vi "Add content to Engine library.vi"(6 "Project Name":string, 8 "error in":errorcluster, 9 "Project Root":path, 10 "CD Wizard - Internal Data":T1, 11 "CD Template":refnum<class "NIVS_CD Template.lvclass">) -> (0 "error out":errorcluster)   [LabVIEW 2020, in "NIVS_CD Template.lvclass"]
doc: "Add all virtual folders and VIs to the Engine library."
uses:
  NIVS_CD Template.lvclass
  NIVS_Consolidated_CDW_MetaDataObj/Internal data.ctl
  NIVS_Consolidated_CDW_MetaDataObj/CD Engine lvlib.ctl
  NIVS_Consolidated_CDW_MetaDataObj/Add Item - Type.ctl
  NIVS_CD Template.lvclass/NIVS_CD Template.ctl
  NIVS_Consolidated_CDW_MetaDataObj/NIVS_Consolidated_CDW_MetaDataObj.lvclass
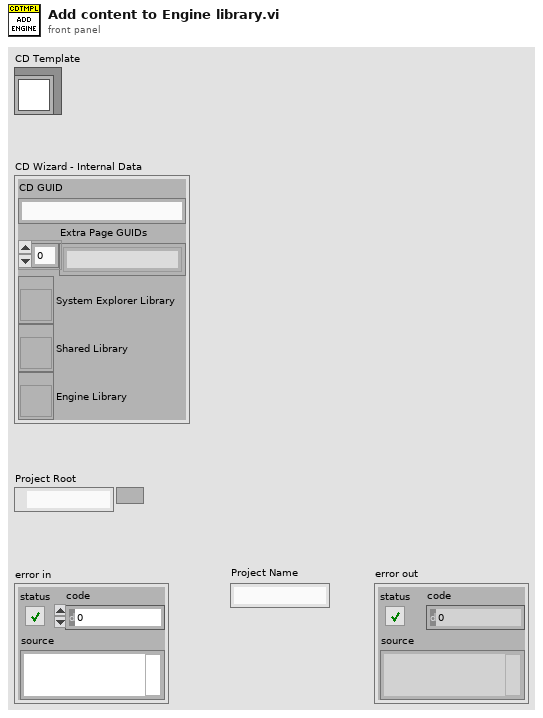
[diagram p1: front panel]
types:
  T1 = typedef "NIVS_Consolidated_CDW_MetaDataObj.lvclass/Internal data.ctl" = cluster{"CD GUID":string, "Extra Page GUIDs":string[], "System Explorer Library":refnum<vi>, "Shared Library":refnum<vi>, "Engine Library":refnum<vi>}
  T2 = typedef "NIVS_Consolidated_CDW_MetaDataObj.lvclass/CD Engine lvlib.ctl" = enum16{"LibraryFileName", "LibraryFolderName", "Engine.FolderName", "Engine.Init.FolderName", "Engine.Run.FolderName", "Engine.Shutdown.FolderName", "Types.FolderName", "Engine.RT Driver VI.TemplatePath", "Engine.RT Driver VI.FileName", "Engine.PPL.RT Driver VI_InlineAsync.FileName", "Engine.RTStateVariables.Name", "Engine.PPL.RTStateVariables.Name", "Engine.RTStateVariables.Name.NoExtension", "Engine.Async.NameExtension", "Engine.Async.TemplateName", "Engine.PPL.Async.TemplateName", "Engine.PPL.Async.InitVSGlobals.Name", "Engine.PPL.RT Driver VI_Inline.FileName", "Engine.LaunchCommandLoop.Name", "Engine.CommandLoop.Name"}
  T3 = typedef "NIVS_Consolidated_CDW_MetaDataObj.lvclass/Add Item - Type.ctl" = string
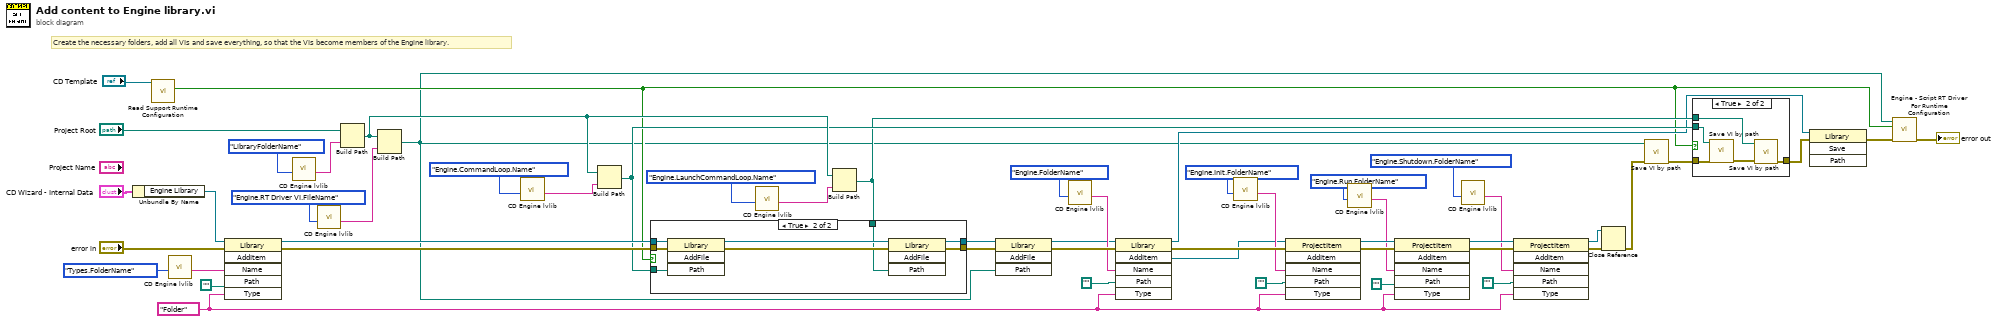
[diagram p0: block diagram]
diagram:
  w21 = T3 "Folder" ("Add Item - Type")
  # "Create the necessary folders, add all VIs and save everything, so that the VIs become members of the Engine library."
  n1 = Unbundle By Name("CD Wizard - Internal Data") -> ("Engine Library"=w33:refnum<vi>)
  n2 = call "Read Support Runtime Configuration.vi"("NIVS_CD Template in"="CD Template") -> ("Support Runtime Configuration"=w4:bool)  [unwired: 8 in, 2 out]
  n3 = call "CD Engine lvlib.vi"("Action"=CD_Engine_lvlib."Types.FolderName") -> ("Output"=w40:string)  [unwired: 10 in]
  n4 = invoke class="Library" method="AddItem"(reference=w33, error in="error in", "Name"=w40, "Path"=path "", "Type"=w21) -> (reference out=w36:refnum<vi>, error out=w51:errorcluster)  [unwired: 1 in, 4 out]
  n5 = call "CD Engine lvlib.vi"("Action"=CD_Engine_lvlib."LibraryFolderName") -> ("Output"=w34:string)  [unwired: 10 in]
  n6 = call "CD Engine lvlib.vi"("Action"=CD_Engine_lvlib."Engine.RT Driver VI.FileName") -> ("Output"=w35:string)  [unwired: 10 in]
  n7 = Build Path(base path="Project Root", name or relative path=w34) -> (appended path=w8:path)
  n8 = Build Path(base path=w8, name or relative path=w35) -> (appended path=w1:path)
  n9 = call "CD Engine lvlib.vi"("Action"=CD_Engine_lvlib."Engine.CommandLoop.Name") -> ("Output"=w11:string)  [unwired: 10 in]
  n10 = Build Path(base path=w8, name or relative path=w11) -> (appended path=w7:path)
  n11 = call "CD Engine lvlib.vi"("Action"=CD_Engine_lvlib."Engine.LaunchCommandLoop.Name") -> ("Output"=w10:string)  [unwired: 10 in]
  n12 = Build Path(base path=w8, name or relative path=w10) -> (appended path=w6:path)
  n13 = case shown="True" w4 {
    tunnel: w51 -> [w56 w64]
    tunnel: w7 -> [_ w61]
    tunnel: w6 -> [_ w59]
    tunnel: [w55 w58] -> w3
    tunnel: [w56 w62] -> w43
    tunnel: w36 -> [w55 w57]
    frame False {
    }
    frame True {
      n14 = invoke class="Library" method="AddFile"(reference=w57, error in=w64, "Path"=w61) -> (reference out=w60:refnum<vi>, error out=w63:errorcluster)  [unwired: 1 in, 2 out]
      n15 = invoke class="Library" method="AddFile"(reference=w60, error in=w63, "Path"=w59) -> (reference out=w58:refnum<vi>, error out=w62:errorcluster)  [unwired: 1 in, 2 out]
    }
  }
  n16 = invoke class="Library" method="AddFile"(reference=w3, error in=w43, "Path"=w1) -> (reference out=w2:refnum<vi>, error out=w42:errorcluster)  [unwired: 1 in, 2 out]
  n17 = call "CD Engine lvlib.vi"("Action"=CD_Engine_lvlib."Engine.FolderName") -> ("Output"=w31:string)  [unwired: 10 in]
  n18 = invoke class="Library" method="AddItem"(reference=w2, error in=w42, "Name"=w31, "Path"=path "", "Type"=w21) -> (reference out=w5:refnum<vi>, error out=w50:errorcluster, "AddItem"=w30:refnum<vi>)  [unwired: 1 in, 3 out]
  n19 = call "CD Engine lvlib.vi"("Action"=CD_Engine_lvlib."Engine.Init.FolderName") -> ("Output"=w37:string)  [unwired: 10 in]
  n20 = invoke class="ProjectItem" method="AddItem"(reference=w30, error in=w50, "Name"=w37, "Path"=path "", "Type"=w21) -> (reference out=w29:refnum<vi>, error out=w49:errorcluster)  [unwired: 1 in, 4 out]
  n21 = call "CD Engine lvlib.vi"("Action"=CD_Engine_lvlib."Engine.Run.FolderName") -> ("Output"=w28:string)  [unwired: 10 in]
  n22 = invoke class="ProjectItem" method="AddItem"(reference=w29, error in=w49, "Name"=w28, "Path"=path "", "Type"=w21) -> (reference out=w25:refnum<vi>, error out=w48:errorcluster)  [unwired: 1 in, 4 out]
  n23 = call "CD Engine lvlib.vi"("Action"=CD_Engine_lvlib."Engine.Shutdown.FolderName") -> ("Output"=w24:string)  [unwired: 10 in]
  n24 = invoke class="ProjectItem" method="AddItem"(reference=w25, error in=w48, "Name"=w24, "Path"=path "", "Type"=w21) -> (reference out=w23:refnum<vi>, error out=w53:errorcluster)  [unwired: 1 in, 4 out]
  n25 = Close Reference(reference=w23, error in (no error)=w53) -> (error out=w52:errorcluster)
  n26 = call "Save VI by path.vi"("error in (no error)"=w52, "VI path"=w1) -> ("error out"=w47:errorcluster)  [unwired: 9 in]
  n27 = case shown="True" w4 {
    tunnel: w47 -> [w65 w70]
    tunnel: [w65 w68] -> w46
    tunnel: w7 -> [_ w67]
    tunnel: w6 -> [_ w66]
    frame False {
    }
    frame True {
      n28 = call "Save VI by path.vi"("error in (no error)"=w70, "VI path"=w67) -> ("error out"=w69:errorcluster)  [unwired: 9 in]
      n29 = call "Save VI by path.vi"("error in (no error)"=w69, "VI path"=w66) -> ("error out"=w68:errorcluster)  [unwired: 9 in]
    }
  }
  n30 = invoke class="Library" method="Save"(reference=w5, error in=w46) -> (error out=w45:errorcluster)  [unwired: 2 in, 3 out]
  n31 = call "Engine - Script RT Driver For Runtime Configuration.vi"("error in"=w45, "Support Runtime Configuration"=w4, "RT Driver VI Path"=w1) -> ("error out"=→"error out":errorcluster)  [unwired: 8 in]
